vi "[ex ce] Methods of point-by-point computation.vi"() -> ()   [LabVIEW 2021]
doc: "<B>Run speed example</B>\n\nThis examlpe compares two methods of calling CalcExpress VI for multiple evaluation of the same formula.\n\n::: CalcExpress Toolkit :::\nCopyright (c) 2000-2026 Konstantin Shifershteyn. All rights reserved."
panel:
  in  "method to call CalcExpress VI":u16(ring) items=["Multiple calls (a call for every data point)", "Single call (using a repeat feature)"]
  in  "Init script":string="ic = 0;                   //initial condition\nfc = 0;                   //final condition\ndt = 10/size(data);       //delta t\nx = vector(ic, data, fc); //data + conditions\ny = data * 0;             //output array\ni = 0;                    //index in y\nj = 1;                    //index in x\nk = 0;                    //temporal variable" caption="script to prepare evaluation (declares and initializes variables)"
  out "Graph":cluster{dbl, dbl, "value out":dbl[]}[](graph)
  out "exec time, ms":u32
  in  "Exec script":string="// performs the discrete integration\nk   += x[j-1] + 4*x[j] + x[j+1];\ny[i] = k/6 * dt;\ni+=1; j+=1;\n" caption="script performing evaluation"
  in  "n points":i32=10000
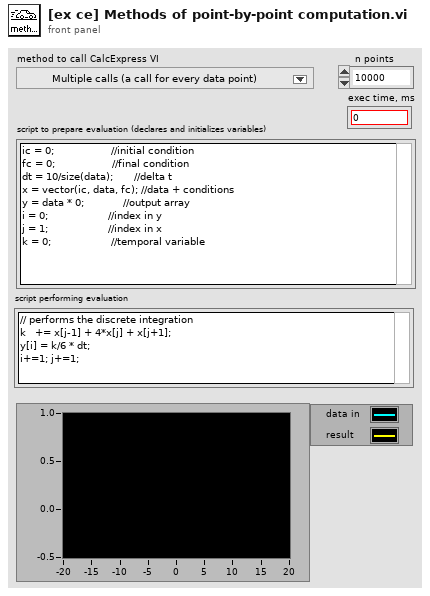
[diagram p1: front panel]
types:
  T1 = enum16{"create", "destroy", "set value", "get value"}
  T2 = typedef "VarMan Variable Context Handle.ctl" = i32
  T3 = typedef "CalcExpress Instance RefNum.ctl" = refnum<k1>
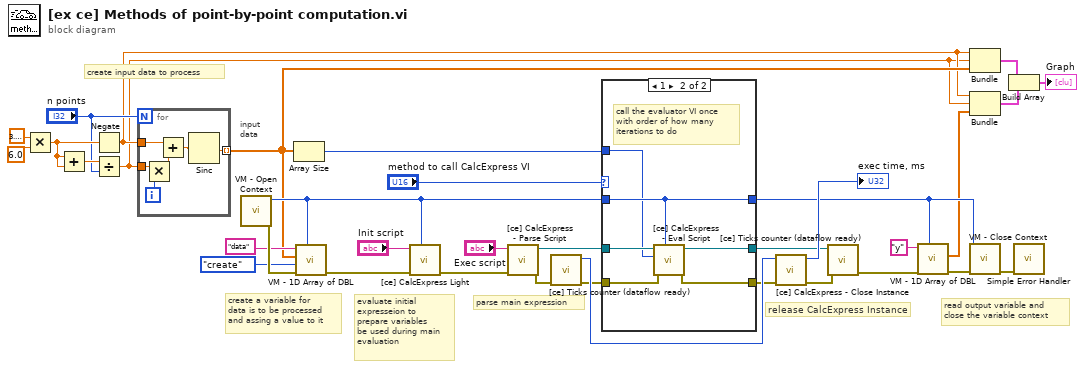
[diagram p0: block diagram]
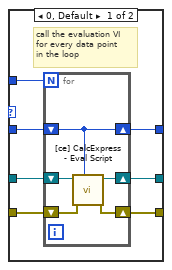
[diagram p2: hidden frame]
diagram:
  # "read output variable and\nclose the variable context"
  # "release CalcExpress Instance"
  # "parse main expression"
  # "evaluate initial\nexpresseion to\nprepare variables\nbe used during main\nevaluation"
  # "create input data to process"
  # "create a variable for\ndata is to be processed\nand assing a value to it"
  # "input\ndata"
  n1 = Multiply(x=3.141592653589793, y=6.0) -> (x*y=w26:dbl)
  n2 = Add(x=w26, y=w26) -> (x+y=w28:dbl)
  n3 = Negate(x=w26) -> (-x=w3:dbl)
  n4 = Divide(x=w28, y="n points") -> (x/y=w2:dbl)
  n5 = for {
    N: "n points" -> [_]
    tunnel: [w40] -> w4 mode=indexing
    tunnel: w2 -> [w37]
    tunnel: w3 -> [w36]
    i -> [w41]
    n6 = Multiply(x=w37, y=w41) -> (x*y=w38:dbl)
    n7 = Add(x=w36, y=w38) -> (x+y=w39:dbl)
    n8 = Sinc(1:w39) -> (0:w40:dbl)
  }
  n9 = call "VM - Open Context.vi"() -> ("error out"=w34:errorcluster, "VC Handle out"=w21:T2)  [unwired: 9 in, 1 out]
  n10 = Array Size(array=w4) -> (size(s)=w13:i32)
  n11 = call "VM - 1D Array of DBL.vi"("VC Handle"=w21, "error in"=w34, "cmd"=T1."create", "value in"=w4, "name_spec"="data" ("name in")) -> ("error out"=w23:errorcluster)  [unwired: 1 in, 5 out]
  n12 = call "[ce] CalcExpress Light.vi"("VC Handle"=w21, "error in"=w23, "expression"="Init script") -> ("error out"=w19:errorcluster)  [unwired: 6 in, 2 out]
  n13 = call "[ce] CalcExpress - Parse Script.vi"("error in"=w19, "expression"="Exec script") -> ("error out"=w18:errorcluster, "CE InstanceRef"=w31:T3)  [unwired: 4 in, 2 out]
  n14 = call "[ce] Ticks counter (dataflow ready).vi"("error in"=w18) -> ("error out"=w17:errorcluster, "ticks (current-input)"=w30:u32)  [unwired: 4 in, 3 out]
  n15 = case shown="1" "method to call CalcExpress VI" {
    tunnel: w13 -> [w48 w54]
    tunnel: [w47 w59] -> w9
    tunnel: w21 -> [w46 w59]
    tunnel: [w45 w58] -> w15
    tunnel: w17 -> [w42 w57]
    tunnel: [w44 w56] -> w16
    tunnel: w31 -> [w43 w55]
    frame 0, Default {
      # "call the evaluation VI\nfor every data point\nin the loop"
      n16 = for {
        N: w48 -> [_]
        shift-right: [w50] -> w44
        shift-left: w42 -> [w53]
        shift-right: [w51] -> w45
        shift-left: w43 -> [w52]
        shift-right: [w49] -> w47
        shift-left: w46 -> [w49]
        n17 = call "[ce] CalcExpress - Eval Script.vi"("VC Handle"=w49, "error in"=w53, "CE InstanceRef"=w52) -> ("error out"=w50:errorcluster, "dup CE InstanceRef"=w51:T3)  [unwired: 2 in, 3 out]
      }
    }
    frame 1 {
      # "call the evaluator VI once\nwith order of how many\niterations to do"
      n18 = call "[ce] CalcExpress - Eval Script.vi"("VC Handle"=w59, "error in"=w57, "repeat (1)"=w54, "CE InstanceRef"=w55) -> ("error out"=w56:errorcluster, "dup CE InstanceRef"=w58:T3)  [unwired: 1 in, 3 out]
    }
  }
  n19 = call "[ce] Ticks counter (dataflow ready).vi"("error in"=w16, "ticks in"=w30) -> ("error out"=w12:errorcluster, "ticks (current-input)"=→"exec time, ms":u32)  [unwired: 3 in, 3 out]
  n20 = call "[ce] CalcExpress - Close Instance.vi"("error in"=w12, "CE InstanceRef"=w15) -> ("error out"=w11:errorcluster)  [unwired: 5 in, 2 out]
  n21 = call "VM - 1D Array of DBL.vi"("VC Handle"=w9, "error in"=w11, "name_spec"="y" ("name in")) -> ("error out"=w10:errorcluster, "value out"=w7:dbl[])  [unwired: 3 in, 4 out]
  n22 = Bundle(w3, w2, w4) -> (w5:cluster{dbl, dbl, dbl[]})  [unwired: 1 in]
  n23 = Bundle(w3, w2, "value out"=w7) -> (w6:cluster{dbl, dbl, "value out":dbl[]})  [unwired: 1 in]
  n24 = call "VM - Close Context.vi"("error in"=w10, "VC Handle"=w9) -> ("error out"=w8:errorcluster)  [unwired: 8 in, 1 out]
  n25 = Build Array(w5, w6) -> (→"Graph":cluster{dbl, dbl, "value out":dbl[]}[])
  n26 = call <vilib>:"Simple Error Handler.vi"("error in (no error)"=w8) -> ()  [unwired: 4 in, 5 out]
